vi "ASD STD estimation VI.vi"(8 "STD Selection":T2(ring), 9 "STD Cut":i32=15, 11 "BL Substraced raw data":dbl[](array[numeric])) -> (0 "Selected STD (pA)":dbl, 1 "R STD select":string, 3 "STD cluster":T1)   [LabVIEW 2018]
uses:
  <vilib>/Analysis/baseanly.llb/Mean (DBL).vi
  <vilib>/Analysis/baseanly.llb/Unimode.vi
  <vilib>/Analysis/NI_AALBase.lvlib
panel:
  out "mode":dbl caption="モード"
  out "STD Cut 2":i32=15
  out "配列":dbl[](array[numeric])
  out "All STD (pA)":dbl
  out "Div STD Mode (pA)":dbl
  out "Div STD mean (pA)":dbl format="%0.6f"
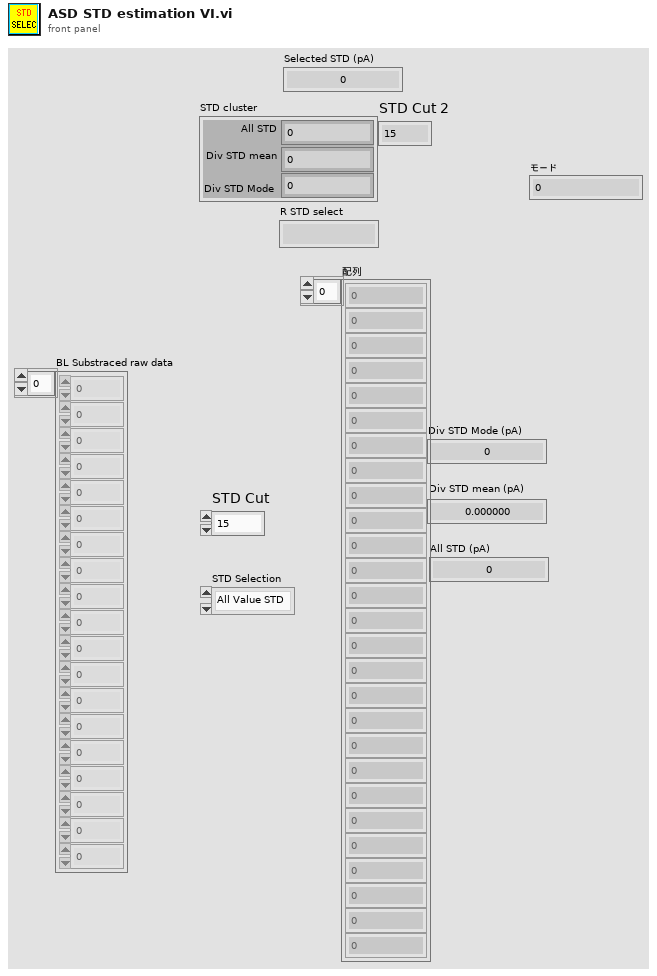
[diagram p1: front panel]
types:
  T1 = cluster{"All STD":dbl, "Div STD mean":dbl, "Div STD Mode":dbl}
  T2 = enum16{"All Value STD", "Div STD Mean STD", "DivSTD Mode STD"}
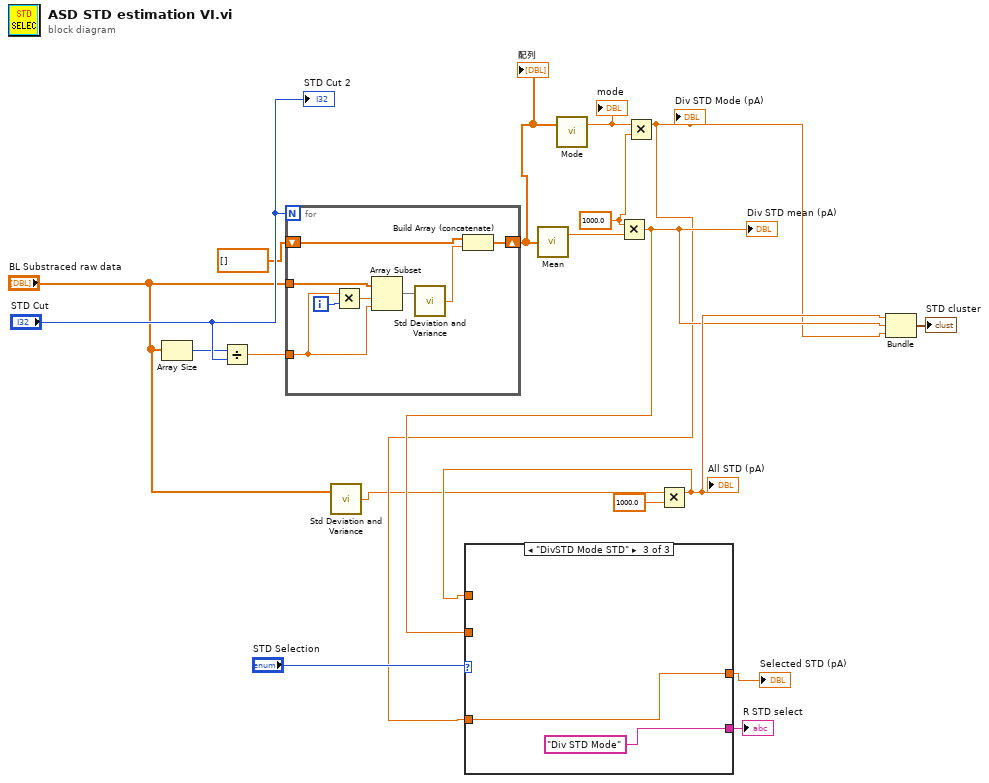
[diagram p0: block diagram]
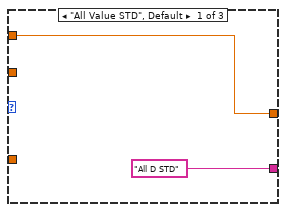
[diagram p2: hidden frame]
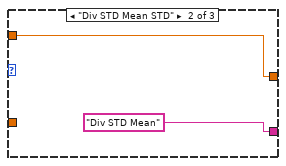
[diagram p3: hidden frame]
diagram:
  w11 = 1000.0 ("x")
  n1 = Array Size(array="BL Substraced raw data") -> (size(s)=w14:i32)
  n2 = Divide(x=w14, y="STD Cut") -> (x/y=w18:dbl)
  n3 = for {
    N: "STD Cut" -> [_]
    tunnel: "BL Substraced raw data" -> [w26]
    tunnel: w18 -> [w25]
    shift-right: [w21] -> w13
    shift-left: dbl[] [] -> [w20]
    i -> [w24]
    n4 = Multiply(x=w25, y=w24) -> (x*y=w23:dbl)
    n5 = Array Subset(array=w26, index=w23, length=w25) -> (w19:dbl[])
    n6 = call <vilib>:"Std Deviation and Variance.vi"("X"=w19) -> ("standard deviation"=w22:dbl)  [unwired: 1 in, 2 out]
    n7 = Build Array (concatenate)(w20, w22) -> (w21:dbl[])
  }
  "配列" <- w13
  n8 = call <vilib>:"Std Deviation and Variance.vi"("X"="BL Substraced raw data") -> ("standard deviation"=w1:dbl)  [unwired: 1 in, 2 out]
  n9 = call-poly <vilib>:"Mean.vi"("X"=w13) -> ("mean"=w15:dbl)  [unwired: 1 out]
  n10 = call-poly <vilib>:"Mode.vi"("X"=w13) -> ("mode"=w12:dbl)  [unwired: 1 in, 1 out]
  "mode" <- w12
  n11 = Multiply(x=w11, y=w15) -> (x*y=w5:dbl)
  "Div STD mean (pA)" <- w5
  n12 = Multiply(x=w12, y=w11) -> (x*y=w4:dbl)
  "Div STD Mode (pA)" <- w4
  n13 = Multiply(x=w1, y=1000.0) -> (x*y=w6:dbl)
  "All STD (pA)" <- w6
  n14 = case shown="\"DivSTD Mode STD\"" "STD Selection" {
    tunnel: w6 -> [w28 _ _]
    tunnel: [w28 w30 w32] -> w7
    tunnel: w5 -> [_ w30 _]
    tunnel: w4 -> [_ _ w32]
    tunnel: ["All D STD" "Div STD Mean" "Div STD Mode"] -> w2
    frame "All Value STD", Default {
    }
    frame "Div STD Mean STD" {
    }
    frame "DivSTD Mode STD" {
    }
  }
  "Selected STD (pA)" <- w7
  "R STD select" <- w2
  n15 = Bundle(w6, w5, w4) -> (→"STD cluster":cluster{dbl, dbl, dbl})  [unwired: 1 in]
  "STD Cut 2" <- "STD Cut"
